vi "eDyno AI Setup.vi"(0 "AI Physical Channel":string="PXI1Slot2/ai0", 1 "AI Range (g)":dbl=50.0, 2 "Sensitivity (mV/g)":dbl=100.0, 3 "Sample Rate (S/s)":dbl=51200.0, 4 "Buffer Samples":i32=51200, 5 "error in":errorcluster) -> (14 "task out":refnum<k21>, 19 "error out":errorcluster)   [LabVIEW 2026]
doc: "Creates the AI acceleration task for the loopback channel: accelerometer channel in g (sensitivity in mV/g), IEPE excitation set to NONE because AI is driven by the AO output, not by a real ICP sensor (switch the excitation constant to Internal / 4 mA when a real 356A15 is connected). Continuous sample clock at Sample Rate, buffer of Buffer Samples. Not started."
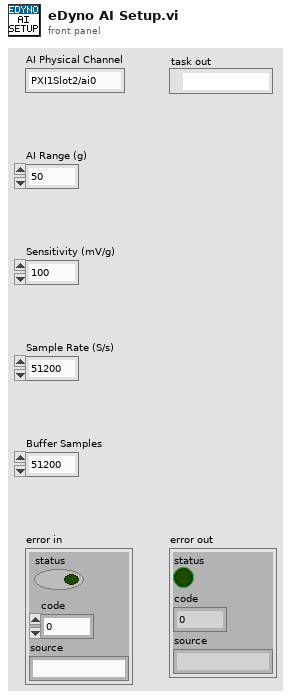
[diagram p1: front panel]
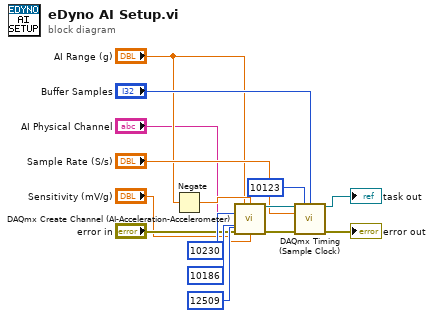
[diagram p0: block diagram]
diagram:
  n1 = Negate(x="AI Range (g)") -> (-x=w9:dbl)
  n2 = call <vilib>:"DAQmx Create Channel (AI-Acceleration-Accelerometer).vi"("maximum value"="AI Range (g)", "minimum value"=w9, "physical channels"="AI Physical Channel", "current excitation source"=10230 ("IEPE Excitation (None for loopback)"), "units"=10186 ("Acceleration Units"), "error in"="error in", "sensitivity"="Sensitivity (mV/g)", "sensitivity units"=12509 ("Sensitivity Units")) -> ("task out"=w14:refnum<k21>, "error out"=w15:errorcluster)  [unwired: 6 in]
  n3 = call <vilib>:"DAQmx Timing (Sample Clock).vi"("task/channels in"=w14, "sample mode"=10123 ("Sample Mode"), "samples per channel"="Buffer Samples", "rate"="Sample Rate (S/s)", "error in"=w15) -> ("task out"=→"task out":refnum<k21>, "error out"=→"error out":errorcluster)  [unwired: 9 in]
